vi "main.vi"() -> ()   [LabVIEW 2016]
uses:
  controls/Level2.ctl
panel:
  in  "StringArray":string[](array[string])
  in  "BooleanArray":bool[](array[boolean])
  in  "NumericArray":dbl[](array[numeric])
  in  "BigCluster":T2
  in  "Cluster":T3
  in  "String":string
  in  "Boolean":bool
  in  "Numeric":dbl
  in  "Tab Control":T4(tab)
  in  "BigCluster":T2
  in  "Cluster":T3
  in  "String":string
  in  "Boolean":bool
  in  "Numeric":dbl
  in  "Time lapse(sec)":u32
  in  "Panel Name":string
  in  "Refresh":bool
  in  "Listbox":i32(listbox)
  in  "Panel Name 2":string
  in  "Listbox 2":i32(listbox)
  in  "Run":bool
  in  "DisableListbox":i32(listbox)
  in  "MultiselectListbox":i32[](listbox)
  in  "Single Listbox":i32(listbox)
  out "Listbox Value":i32
  out "Selected Value":i32[](array[numeric])
  in  "Disabled MC Listbox":i32(listbox)
  in  "Multiselect MC Listbox":i32[](listbox)
  in  "MC Listbox":i32(listbox)
  out "MCListbox Value":i32
  out "MCL Selected Value":i32[](array[numeric])
  in  "Marksheet":string[][](table)=[["", "Class A", "Class B", "Total"], ["Biology", "10", "7", "17"], ["Chemistry", "8", "11", "19"], ["Physics", "12", "14", "26"], ["Total", "30", "32", "62"]]
  in  "Multiselect Tree":string[](tree)
  in  "Tree Control":string(tree)="Kavin"
  out "Item Tag":string
  out "Selected Tags":string[](array[string])
  out "Item Name":string
  in  "OK":bool
  in  "Stop":bool
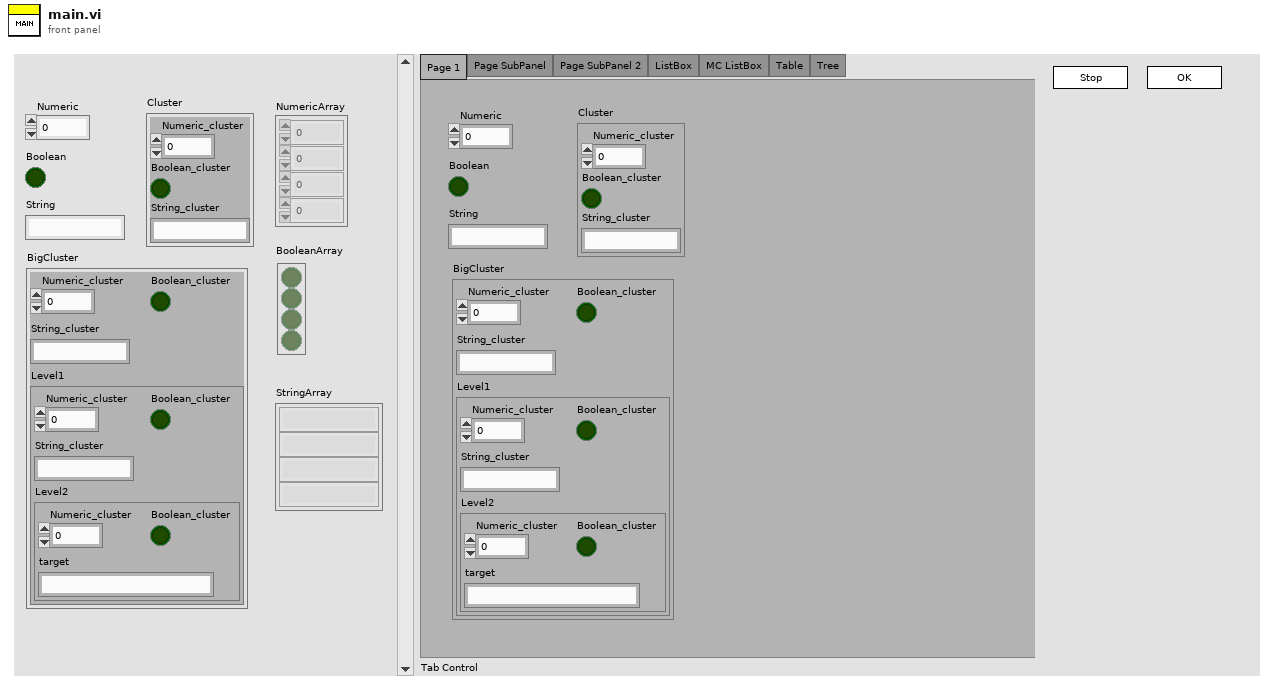
[diagram p1: front panel]
types:
  T1 = typedef "Level2.ctl" = cluster{"Numeric_cluster":dbl, "Boolean_cluster":bool, "target":string}
  T2 = cluster{"Numeric_cluster":dbl, "Boolean_cluster":bool, "String_cluster":string, "Level1":cluster{"Numeric_cluster":dbl, "Boolean_cluster":bool, "String_cluster":string, "Level2":T1}}
  T3 = cluster{"Numeric_cluster":dbl, "Boolean_cluster":bool, "String_cluster":string}
  T4 = enum32{"Page 1", "Page SubPanel", "Page SubPanel 2", "ListBox", "MC ListBox", "Table", "Tree"}
  T5 = enum32{"Invalid", "Standard", "Closed", "Hidden", "Minimized", "Maximized"}
  T6 = enum32{"invalid app kind", "Development System", "Run Time System", "Student Edition", "Embedded LabVIEW", "Evaluation", "Custom"}
  T7 = enum8{"Enabled", "Disabled", "Disabled and Grayed Out"}
  T8 = cluster{"Core":cluster{"Current VI Reference":refnum<vi>, "Close Panel on Exit?":bool}, "VI Name":string, "VI Ref":refnum<vi>, "Panel Folder Path":path, "Time lapse(sec)":u32, "Panel 2 Folder Path":path, "Panel 2 VI ref":refnum<vi>, "VI Running?":bool}
  T9 = cluster{"Current VI Reference":refnum<vi>, "Close Panel on Exit?":bool}
  T10 = enum32{"Bad", "Idle", "Run top level", "Running"}[]
  T11 = enum32{"Bad", "Idle", "Run top level", "Running"}
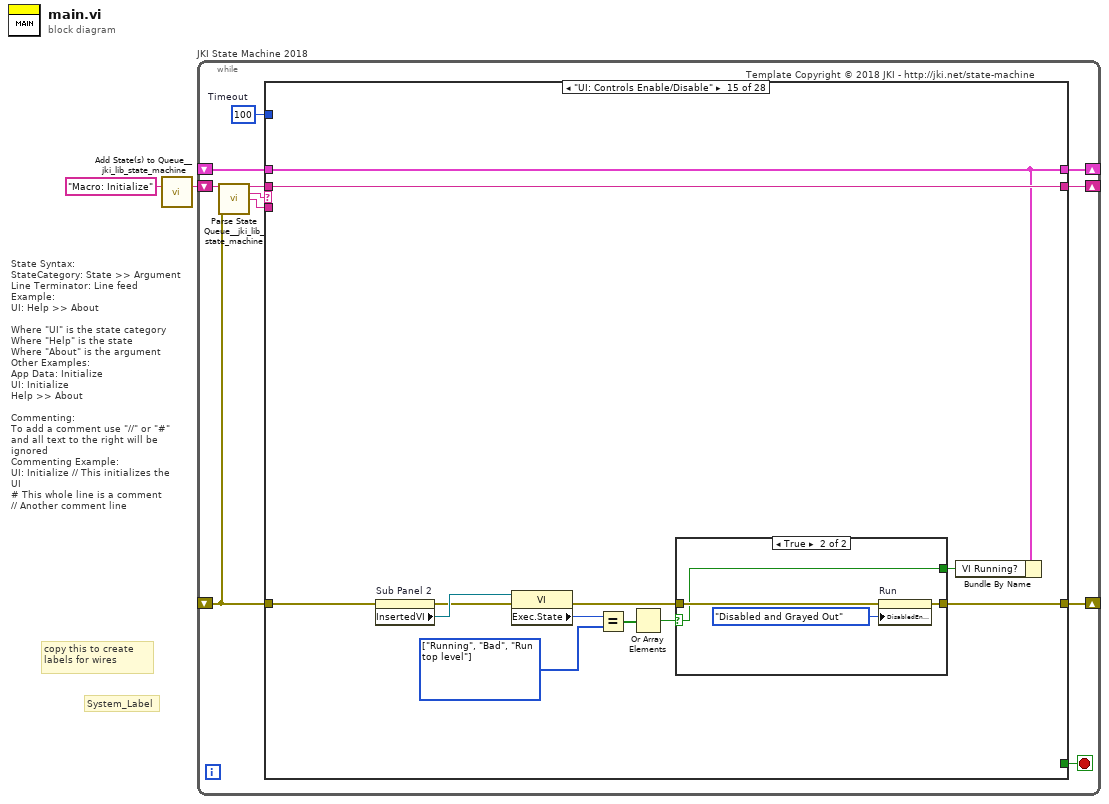
[diagram p0: block diagram]
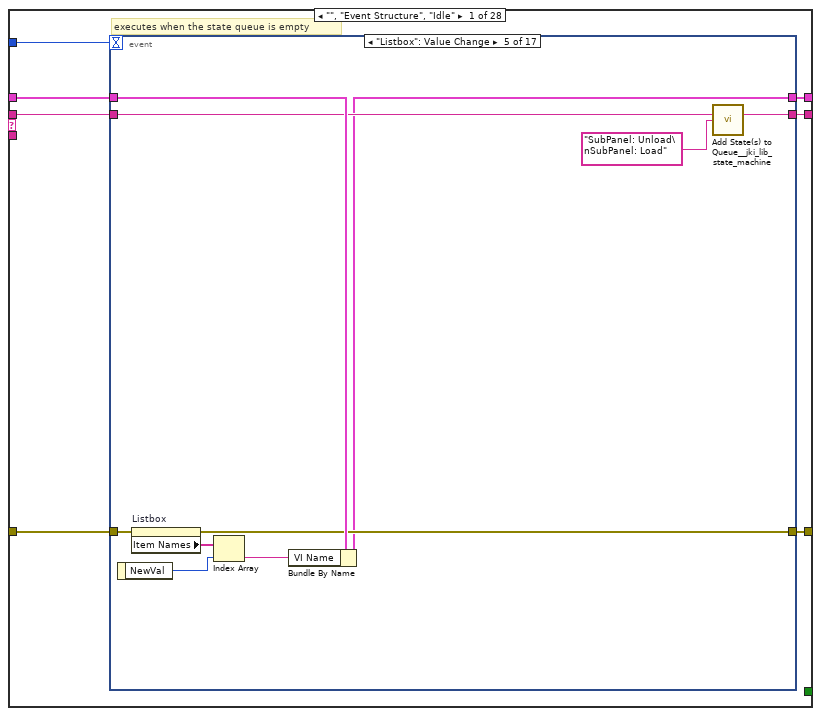
[diagram p2: hidden frame]
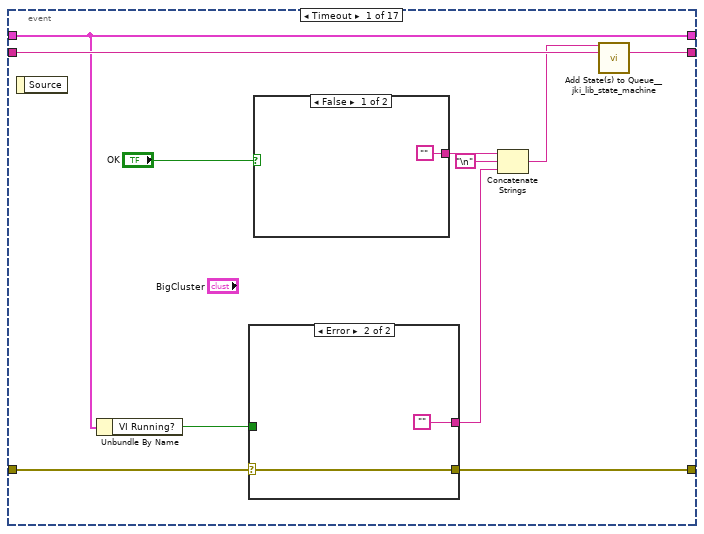
[diagram p3: hidden frame]
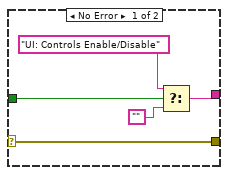
[diagram p4: hidden frame]
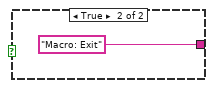
[diagram p5: hidden frame]
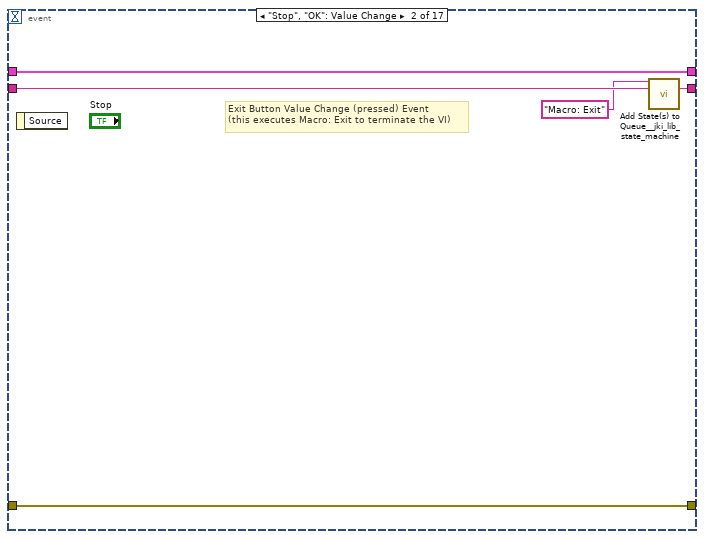
[diagram p6: hidden frame]
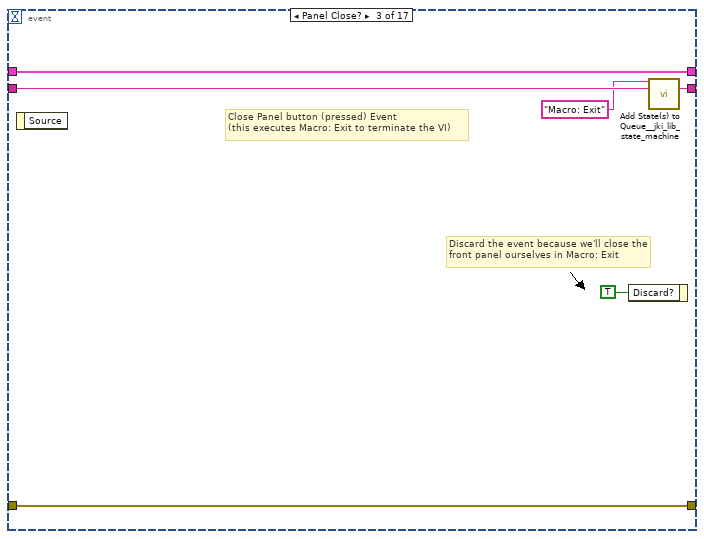
[diagram p7: hidden frame]
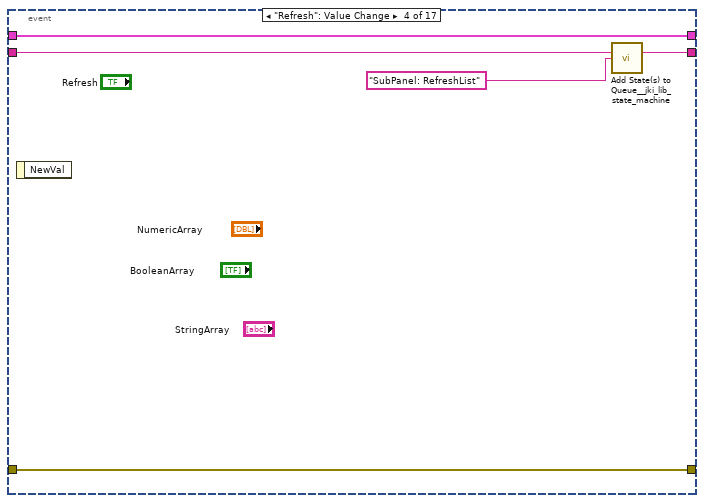
[diagram p8: hidden frame]
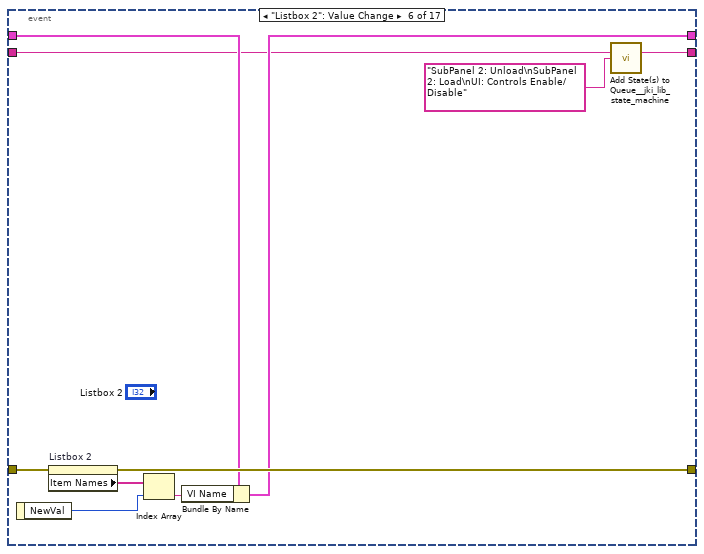
[diagram p9: hidden frame]
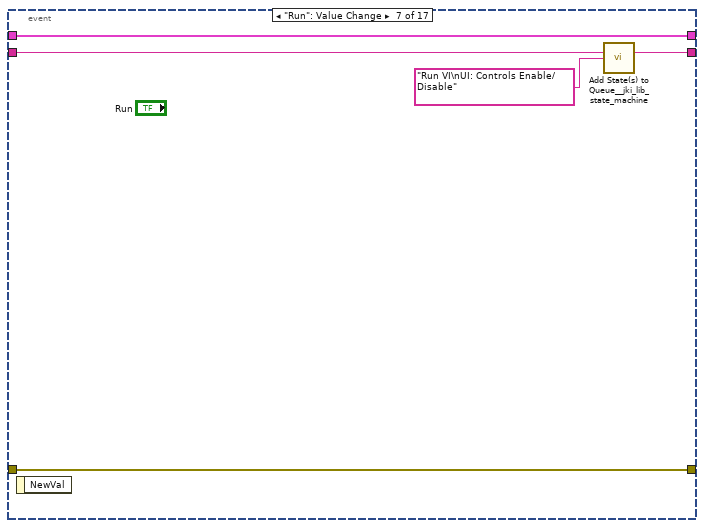
[diagram p10: hidden frame]
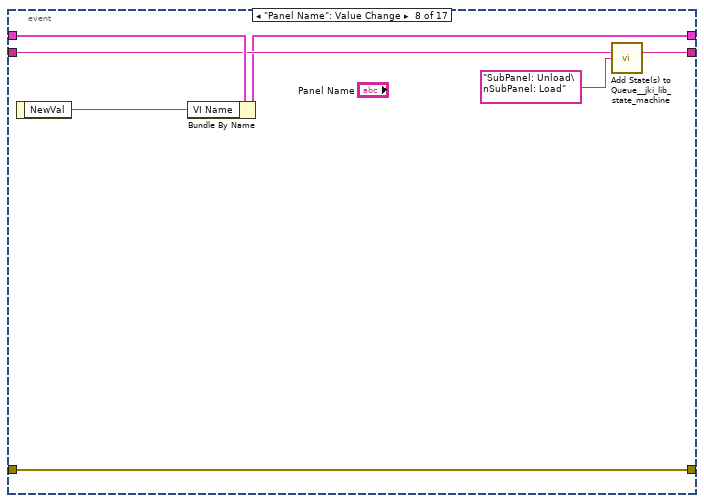
[diagram p11: hidden frame]
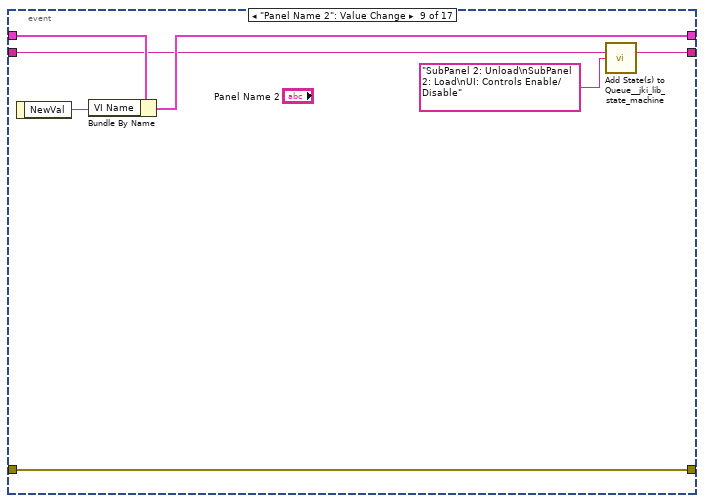
[diagram p12: hidden frame]
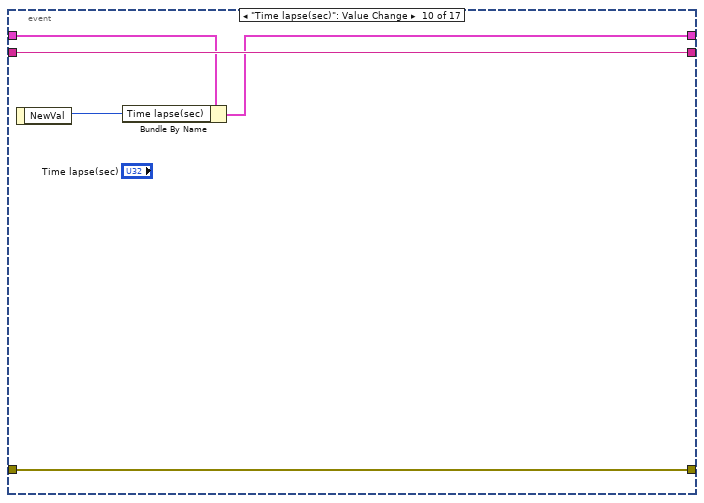
[diagram p13: hidden frame]
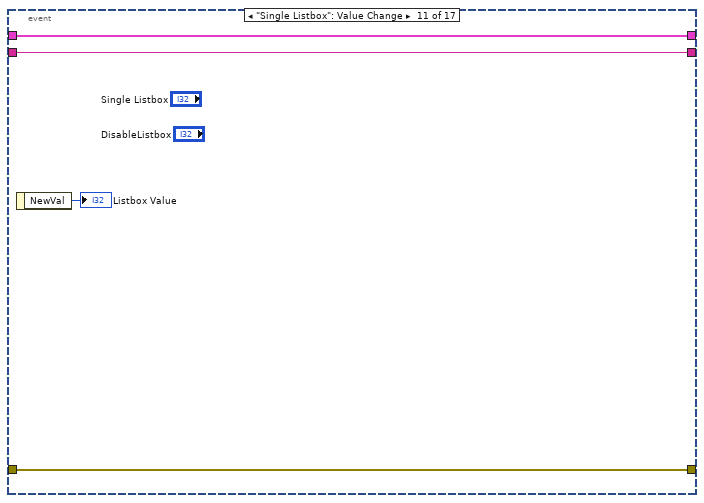
[diagram p14: hidden frame]
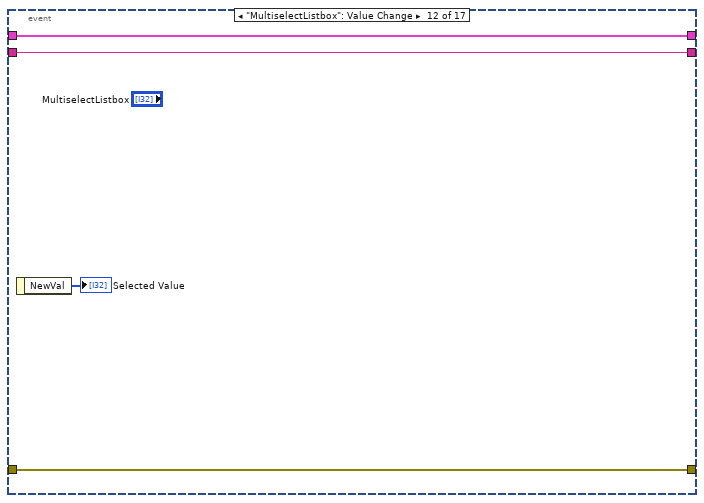
[diagram p15: hidden frame]
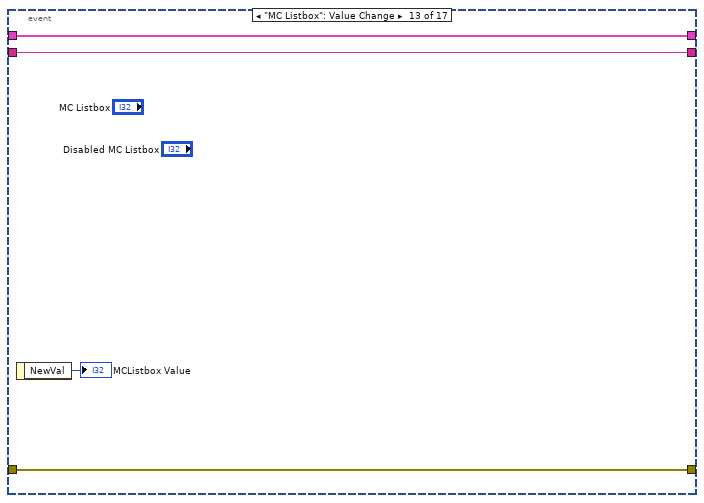
[diagram p16: hidden frame]
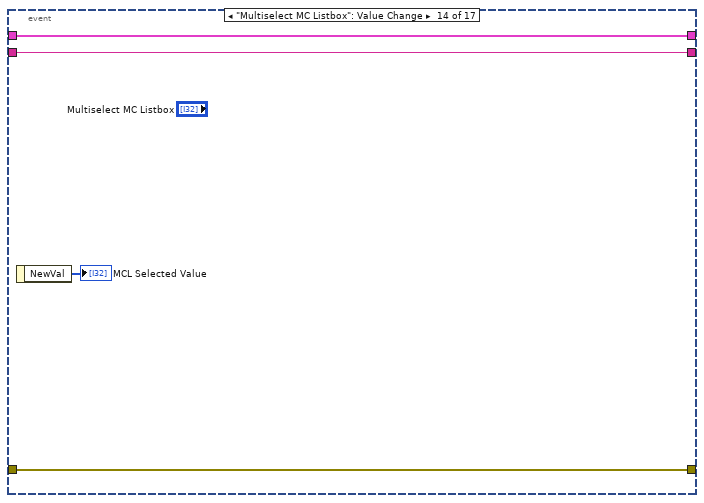
[diagram p17: hidden frame]
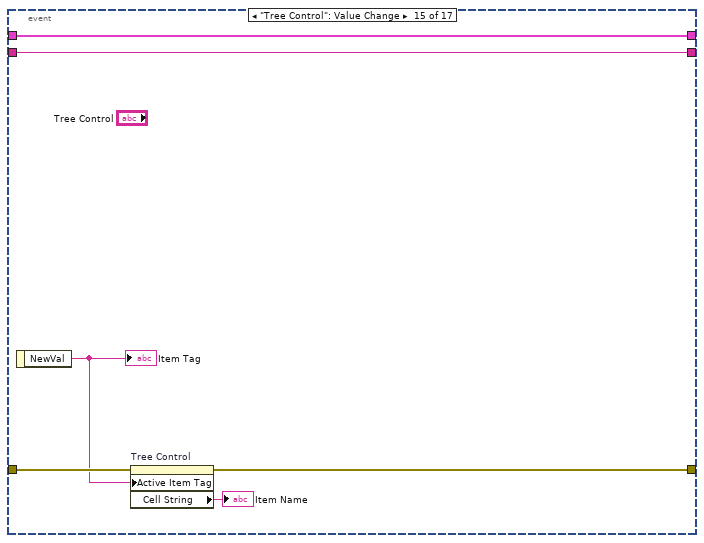
[diagram p18: hidden frame]
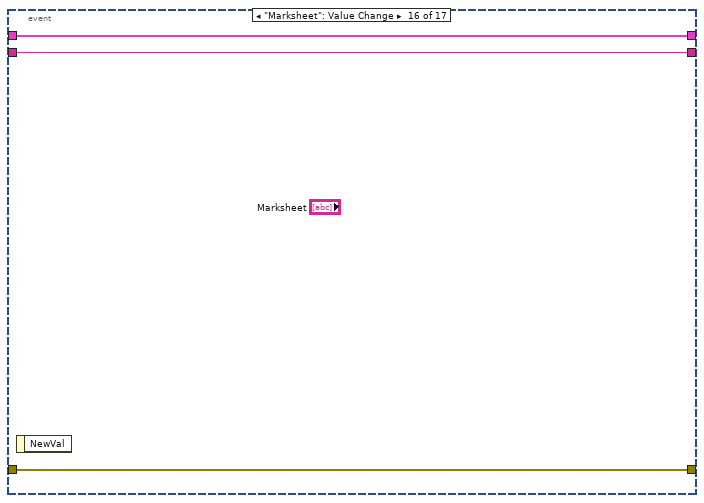
[diagram p19: hidden frame]
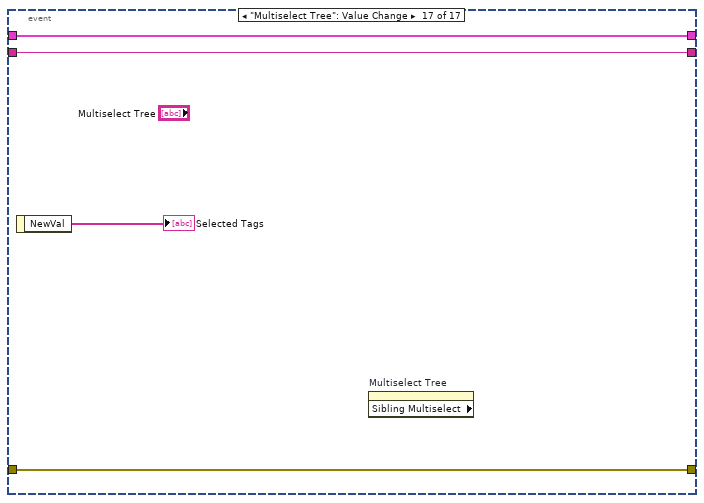
[diagram p20: hidden frame]
diagram:
  # "State Syntax:\nStateCategory: State >> Argument\nLine Terminator: Line feed\nExample:\nUI: Help >> About\n\nWhere \"UI\" is the state category\nWhere \"Help\" is the state\nWhere \"About\" is the argument\nOther Examples:\nApp Data: Initialize\nUI: Initialize\nHelp >> About\n\nCommenting:\nTo add a comment use \"//\" or \"#\" and all text to the right will be ignored\nCommenting Example:\nUI: Initialize // This initializes the UI\n# This whole line is a comment\n// Another comment line"
  # "copy this to create labels for wires"
  # "System_Label"
  n1 = call <vilib>:"Add State(s) to Queue__jki_lib_state_machine.vi"("State(s) in (\"\")"="Macro: Initialize") -> ("States Out"=w2:string)  [unwired: 14 in]
  n2 = while "JKI State Machine 2018" {
    shift-right: [w6] -> _
    shift-left: _ -> [w5]
    shift-right: [w9] -> _
    shift-left: _ -> [w3]
    shift-right: [w8] -> _
    shift-left: w2 -> [w10]
    stop <- w7 stop-if-true
    w4 = 100  # Timeout
    # "Template Copyright © 2018 JKI - http://jki.net/state-machine"
    n3 = call <vilib>:"Parse State Queue__jki_lib_state_machine.vi"("State Queue"=w10, "Error In (no error)"=w3) -> ("Remaining States"=w12:string, "Current State"=w13:string, "Arguments"=w11:string)  [unwired: 11 in]
    n4 = case shown="\"UI: Controls Enable/Disable\"" w13 {
      selector: w13 -> [_ _ w134 _ _ _ _ _ _ _ _ _ _ _ _ _ _ _ _ _ _ _ _ _ _ _ _ _]
      tunnel: w12 -> [w20 w133 w138 w159 w165 w170 w174 w194 w200 w204 w211 w217 w228 w297 w309 w321 w326 w336 w340 w354 w364 w387 w420 w434 w436 w442 w453 w457]
      tunnel: w11 -> [_ _ _ _ _ _ _ _ _ _ _ w212 w222 _ _ _ _ _ _ _ _ _ _ _ _ _ _ _]
      tunnel: w5 -> [w18 w130 w136 w155 w162 w168 w171 _ w195 w201 w209 w215 w224 w295 w298 w318 w323 w333 w337 w349 w361 w382 w418 w426 w435 w440 w450 w454]
      tunnel: [w17 w131 w140 w147 errorcluster {"status"=FALSE, "code"=0, "source"=""} ("error out") w167 w172 w175 w196 w202 w206 w213 w225 w294 w300 w319 w324 w334 w338 w342 w355 w385 w416 w428 w437 w439 w451 w455] -> w9
      tunnel: w3 -> [w16 w131 w139 w149 w161 w167 w172 w176 w197 w202 w208 w214 w226 w294 w301 w319 w324 w334 w338 w352 w357 w379 w419 w429 w437 w441 w451 w455]
      tunnel: [w19 w132 w137 w158 w164 w169 w173 w193 w199 w203 w210 w216 w227 w296 w309 w320 w325 w335 w339 w353 w363 w386 w420 w434 w436 w442 w452 w456] -> w8
      tunnel: [_ _ _ _ _ TRUE _ _ _ _ _ _ _ _ _ _ _ _ _ _ _ _ _ _ _ _ _ _] -> w7
      tunnel: [w15 w130 w136 w157 w162 w168 w171 w188 w195 w201 w209 w215 w224 w295 w298 w318 w323 w333 w337 w349 w361 w381 w418 w425 w435 w438 w450 w454] -> w6
      tunnel: w4 -> [w14 _ _ _ _ _ _ _ _ _ _ _ _ _ _ _ _ _ _ _ _ _ _ _ _ _ _ _]
      frame "", "Event Structure", "Idle" {
        # "executes when the state queue is empty"
        n5 = event shown="[4] \"Listbox\": Value Change" {
          selector: _ -> [_ _ _ _ _ _ _ _ _ _ _ _ _ _ _ _ _]
          dyn-events: _ -> [_ _ _ _ _ _ _ _ _ _ _ _ _ _ _ _ _]
          timeout: w14 -> [_ _ _ _ _ _ _ _ _ _ _ _ _ _ _ _ _]
          tunnel: w20 -> [w31 w45 w51 w54 w65 w68 w79 w87 w90 w100 w104 w108 w112 w116 w122 w125 w129]
          tunnel: [w30 w44 w50 w53 w64 w67 w78 w86 w89 w100 w104 w108 w112 w116 w122 w125 w129] -> w19
          tunnel: w18 -> [w28 w42 w48 w55 w66 w71 w80 w88 w93 w97 w102 w106 w110 w114 w121 w123 w127]
          tunnel: [w21 w43 w49 w56 w61 w74 w81 w84 w95 w99 w103 w107 w111 w115 w119 w124 w128] -> w17
          tunnel: w16 -> [w22 w43 w49 w56 w62 w75 w81 w84 w95 w99 w103 w107 w111 w115 w120 w124 w128]
          tunnel: [w28 w42 w48 w55 w58 w70 w80 w82 w92 w96 w102 w106 w110 w114 w121 w123 w127] -> w15
          event Timeout {
            n6 = event-data() -> ()  [unwired: 1 in, 1 out]
            n7 = Unbundle By Name(w28) -> ("VI Running?"=w27:bool)
            n8 = case shown="Error" w22 {
              selector: w22 -> [w32 w37]
              tunnel: [w33 ""] -> w26
              tunnel: w27 -> [w36 _]
              tunnel: [w32 w37] -> w21
              frame No Error {
                n9 = Select(t="UI: Controls Enable/Disable", s=w36, f="") -> (s? t:f=w33:string)
              }
              frame Error {
              }
            }
            n10 = case shown="False" "OK" {
              tunnel: ["" "Macro: Exit"] -> w25
              frame False {
              }
              frame True {
              }
            }
            n11 = Concatenate Strings(w25, "\n", w26) -> (w23:string)
            n12 = call <vilib>:"Add State(s) to Queue__jki_lib_state_machine.vi"("State(s) in Front (\"\")"=w23, "State(s) in (\"\")"=w31) -> ("States Out"=w30:string)  [unwired: 13 in]
          }
          event "Stop", "OK": Value Change {
            # "Exit Button Value Change (pressed) Event\n(this executes Macro: Exit to terminate the VI)"
            n13 = event-data() -> ()  [unwired: 1 in, 1 out]
            n14 = call <vilib>:"Add State(s) to Queue__jki_lib_state_machine.vi"("State(s) in Front (\"\")"="Macro: Exit", "State(s) in (\"\")"=w45) -> ("States Out"=w44:string)  [unwired: 13 in]
          }
          event Panel Close? {
            # "Discard the event because we'll close the front panel ourselves in Macro: Exit"
            # "Close Panel button (pressed) Event\n(this executes Macro: Exit to terminate the VI)"
            n15 = event-data() -> ()  [unwired: 1 in, 1 out]
            n16 = event-data("Discard?"=TRUE) -> ()  [unwired: 1 in, 1 out]
            n17 = call <vilib>:"Add State(s) to Queue__jki_lib_state_machine.vi"("State(s) in Front (\"\")"="Macro: Exit", "State(s) in (\"\")"=w51) -> ("States Out"=w50:string)  [unwired: 13 in]
          }
          event "Refresh": Value Change {
            n18 = event-data() -> ()  [unwired: 1 in, 1 out]
            n19 = call <vilib>:"Add State(s) to Queue__jki_lib_state_machine.vi"("State(s) in (\"\")"=w54, "State(s) at Back (\"\")"="SubPanel: RefreshList") -> ("States Out"=w53:string)  [unwired: 13 in]
          }
          event "Listbox": Value Change {
            n20 = event-data() -> ("NewVal"=w59:i32)  [unwired: 1 in]
            n21 = property on="Listbox" class="LstBox (strict)"(error in=w62) -> (error out=w61:errorcluster, "Item Names"=w60:string[])  [unwired: 1 in, 1 out]
            n22 = Index Array(array=w60, index=w59) -> (element=w57:string)
            n23 = Bundle By Name(cluster=w66, "VI Name"=w57) -> (w58:T8)
            n24 = call <vilib>:"Add State(s) to Queue__jki_lib_state_machine.vi"("State(s) in (\"\")"=w65, "State(s) at Back (\"\")"="SubPanel: Unload\nSubPanel: Load") -> ("States Out"=w64:string)  [unwired: 13 in]
          }
          event "Listbox 2": Value Change {
            n25 = event-data() -> ("NewVal"=w73:i32)  [unwired: 1 in]
            n26 = property on="Listbox 2" class="LstBox (strict)"(error in=w75) -> (error out=w74:errorcluster, "Item Names"=w76:string[])  [unwired: 1 in, 1 out]
            n27 = Index Array(array=w76, index=w73) -> (element=w72:string)
            n28 = Bundle By Name(cluster=w71, "VI Name"=w72) -> (w70:T8)
            n29 = call <vilib>:"Add State(s) to Queue__jki_lib_state_machine.vi"("State(s) in (\"\")"=w68, "State(s) at Back (\"\")"="SubPanel 2: Unload\nSubPanel 2: Load\nUI: Controls Enable/Disable") -> ("States Out"=w67:string)  [unwired: 13 in]
          }
          event "Run": Value Change {
            n30 = event-data() -> ()  [unwired: 1 in, 1 out]
            n31 = call <vilib>:"Add State(s) to Queue__jki_lib_state_machine.vi"("State(s) in (\"\")"=w79, "State(s) at Back (\"\")"="Run VI\nUI: Controls Enable/Disable" ("State(s) at Back (\"\")")) -> ("States Out"=w78:string)  [unwired: 13 in]
          }
          event "Panel Name": Value Change {
            n32 = event-data() -> ("NewVal"=w83:string)  [unwired: 1 in]
            n33 = Bundle By Name(cluster=w88, "VI Name"=w83) -> (w82:T8)
            n34 = call <vilib>:"Add State(s) to Queue__jki_lib_state_machine.vi"("State(s) in (\"\")"=w87, "State(s) at Back (\"\")"="SubPanel: Unload\nSubPanel: Load") -> ("States Out"=w86:string)  [unwired: 13 in]
          }
          event "Panel Name 2": Value Change {
            n35 = event-data() -> ("NewVal"=w94:string)  [unwired: 1 in]
            n36 = Bundle By Name(cluster=w93, "VI Name"=w94) -> (w92:T8)
            n37 = call <vilib>:"Add State(s) to Queue__jki_lib_state_machine.vi"("State(s) in (\"\")"=w90, "State(s) at Back (\"\")"="SubPanel 2: Unload\nSubPanel 2: Load\nUI: Controls Enable/Disable") -> ("States Out"=w89:string)  [unwired: 13 in]
          }
          event "Time lapse(sec)": Value Change {
            n38 = event-data() -> ("NewVal"=w98:u32)  [unwired: 1 in]
            n39 = Bundle By Name(cluster=w97, "Time lapse(sec)"=w98) -> (w96:T8)
          }
          event "Single Listbox": Value Change {
            n40 = event-data() -> ("NewVal"=→"Listbox Value":i32)  [unwired: 1 in]
          }
          event "MultiselectListbox": Value Change {
            n41 = event-data() -> ("NewVal"=→"Selected Value":i32[])  [unwired: 1 in]
          }
          event "MC Listbox": Value Change {
            n42 = event-data() -> ("NewVal"=→"MCListbox Value":i32)  [unwired: 1 in]
          }
          event "Multiselect MC Listbox": Value Change {
            n43 = event-data() -> ("NewVal"=→"MCL Selected Value":i32[])  [unwired: 1 in]
          }
          event "Tree Control": Value Change {
            n44 = event-data() -> ("NewVal"=w118:string)  [unwired: 1 in]
            "Item Tag" <- w118
            n45 = property on="Tree Control" class="Tree (strict)"(error in=w120, "Active Item Tag"=w118) -> (error out=w119:errorcluster, "Cell String"=→"Item Name":string)  [unwired: 1 in, 1 out]
          }
          event "Marksheet": Value Change {
            n46 = event-data() -> ()  [unwired: 1 in, 1 out]
          }
          event "Multiselect Tree": Value Change {
            n47 = event-data() -> ("NewVal"=→"Selected Tags":string[])  [unwired: 1 in]
            n48 = property on="Multiselect Tree" class="Tree (strict)" props=["Sibling Multiselect"]() -> ()  [unwired: 2 in, 3 out]
          }
        }
      }
      frame "---------- Core ----------" {
        # "Do not put any code in this frame.\n(it is a separator no-op)"
        n49 = call <vilib>:"Add State(s) to Queue__jki_lib_state_machine.vi"("State(s) in (\"\")"=w133) -> ("States Out"=w132:string)  [unwired: 14 in]
      }
      frame Default {
        w143 = 42 items=["No error", "Argument error", "Memory is full", "Out of zone", "End of file", "File already open", "Generic file I/O error", "File not found", "File permission error", "Disk is full", "Duplicate path", "Too many files open", "System feature not enabled", "Resource file not found", "Cannot add resource", "Resource not found", "Image not found", "Image memory error", "Pen does not exist", "Config type invalid", "Config token not found", "Config parse error", "Config memory error", "Bad external code format", "Bad external code offset", "External code not present", "Null window", "Destroy window error", "Null menu", "Print aborted", "Bad print record", "Print driver error", "Windows error during printing", "Memory error during printing", "Print dialog error", "Generic print error", "Invalid device refnum", "Device not found", "Device parameter error", "Device unit error", "Cannot open device", "Device call aborted", "Generic error", "Cancelled by user", "Object ID too low", "Object ID too high", "Object not in heap", "Unknown heap", "Unknown object (invalid DefProc)", "Unknown object (DefProc not in table)", "Message out of range", "Invalid (null) method", "Unknown message", "Manager call not supported", "Bad address", "Network operation in progress", "Network operation timed out", "Connection is busy", "Network attribute not supported", "Network error", "Address in use", "System out of memory", "Connection aborted", "Connection refused", "Not connected", "Already connected", "Connection closed", "Initialization error (interapplication manager)", "Bad occurrence", "Wait on unbound occurrence handler", "Occurrence queue overflow", "Datalog type conflict", "Unused", "Unrecognized type (interapplication manager)", "Memory corrupt", "Failed to make temporary DLL", "Old CIN version", "Drag socket not found", "Failed to load drop-object", "Failed to register OLE object", "Failed to release OLE object", "Format specifier type mismatch", "Unknown format specifier", "Too few format specifiers", "Too many format specifiers", "Scan failed", "Newer CIN version", "Error converting to variant", "Runtime menu error", "Password tampered", "Variant attribute not found", "Incompatible variant data type", "Event data is not available", "Event Store is not present", "Occurrence is not found", "Event Queue is not created", "Event info is not available", "Refnum passed is NULL", "Error retrieving Class GUID", "Error retrieving CoClass GUID", "Error retrieving TypeLib GUID.", "Bad built application magic bytes.", "Specific driver is different from the specific driver associated with the Logical Name.", "There is no session opened to the class driver.", "Max Error", "MAX - Error with config objects", "MAX - Error loading configuration", "MAX - Group not supported"]
        # "Current State"
        # "Do not delete, rename, or modify this frame.\n(this is used to capture unhandled states and typos)"
        # "Handle mistyped state name (developer tool)"
        n50 = Format Into String(format string="Software Exception: Unhandled State \"%s\"." ("message"), error in=w139, w134) -> (resulting string=w142:string, error out=w141:errorcluster)  [unwired: 1 in]
        n51 = call <vilib>:"Error Cluster From Error Code.vi"("show call chain? (False)"=TRUE, "error in (no error)"=w141, "error message (\"\")"=w142, "error code (0)"=w143) -> ("error out"=w140:errorcluster)  [unwired: 5 in]
        n52 = call <vilib>:"Add State(s) to Queue__jki_lib_state_machine.vi"("State(s) in (\"\")"=w138) -> ("States Out"=w137:string)  [unwired: 14 in]
      }
      frame "Initialize Core Data" {
        # "Do not delete, rename, or modify this frame.\n(this is used to determine panel behavior on exit)"
        # "originally closed?"
        # "exe?"
        # "If panel starts closed or is an EXE, then close it when we exit"
        n53 = property class="VI"(error in=w149) -> (error out=w148:errorcluster, "FP.State"=w152:T5)  [unwired: 1 in, 1 out]
        n54 = property class="App"(error in=w148) -> (error out=w147:errorcluster, "App.Kind"=w146:T6)  [unwired: 1 in, 1 out]
        n55 = control-ref of="Current VI Reference"() -> (w153:refnum<vi>)
        n56 = Equal?(x=w152, y=T5."Closed" ("Front Panel Window:State")) -> (x = y?=w150:bool)
        n57 = Equal?(x=T6."Run Time System" ("Application:Kind"), y=w146) -> (x = y?=w156:bool)
        n58 = Or(x=w150, y=w156) -> (x .or. y?=w154:bool)
        n59 = Bundle By Name(cluster=w155, "Core.Current VI Reference"=w153, "Core.Close Panel on Exit?"=w154) -> (w157:T8)
        n60 = call <vilib>:"Add State(s) to Queue__jki_lib_state_machine.vi"("State(s) in (\"\")"=w159) -> ("States Out"=w158:string)  [unwired: 14 in]
      }
      frame "Error Handler" {
        # "Unhandled Error -- Display it"
        # "Handle any errors here.\nYou can also output any states to clean-up after errors occur"
        # "Clear error"
        n61 = call <vilib>:"General Error Handler.vi"("error in (no error)"=w161) -> ()  [unwired: 10 in, 5 out]
        n62 = call <vilib>:"Add State(s) to Queue__jki_lib_state_machine.vi"("State(s) in Front (\"\")"="/* Post Error States", "State(s) in (\"\")"=w165) -> ("States Out"=w164:string)  [unwired: 13 in]
      }
      frame "Exit" {
        # "Do not put any code in this frame.\n(No errors that occur here will be handled.)"
        n63 = call <vilib>:"Add State(s) to Queue__jki_lib_state_machine.vi"("State(s) in (\"\")"=w170) -> ("States Out"=w169:string)  [unwired: 14 in]
      }
      frame "---------- Data ----------" {
        # "Do not put any code in this frame.\n(It is a separator no-op. You can make a copy of this frame to create a new Data frame)"
        n64 = call <vilib>:"Add State(s) to Queue__jki_lib_state_machine.vi"("State(s) in (\"\")"=w174) -> ("States Out"=w173:string)  [unwired: 14 in]
      }
      frame "Data: Initialize" {
        w182 = FALSE  # VI Running?
        w183 = refnum<vi> refnum  # Panel 2 VI ref
        w185 = path ""  # Panel 2 Folder Path
        w186 = u32 0  # Time lapse(sec)
        w187 = refnum<vi> refnum  # VI Ref
        w189 = path ""  # Panel Folder Path
        w190 = T9 {"Current VI Reference"=refnum, "Close Panel on Exit?"=FALSE}  # Core
        w191 = ""  # VI Name
        # "Initialize the shift-register data, here.\n(data names are defined by what you wire into the bundle function)"
        n65 = vi-ref "_Template.vi"() -> (w179:refnum<vi>)
        n66 = property class="VI"(reference=w179, error in=w176) -> (error out=w175:errorcluster, "Path"=w178:path)  [unwired: 1 out]
        n67 = Strip Path(path=w178) -> (stripped path=w177:path)  [unwired: 1 out]
        n68 = Bundle("Core"=w190, "VI Name"=w191, "VI Ref"=w187, "Panel Folder Path"=w189, "Time lapse(sec)"=w186, "Panel 2 Folder Path"=w185, "Panel 2 VI ref"=w183, "VI Running?"=w182) -> (w192:T8)  [unwired: 1 in]
        n69 = Strip Path(path=w177) -> (stripped path=w181:path)  [unwired: 1 out]
        n70 = Build Path(base path=w181, name or relative path="ExecPanels") -> (appended path=w184:path)
        n71 = Bundle By Name(cluster=w192, "Panel Folder Path"=w177, "Panel 2 Folder Path"=w184) -> (w188:T8)
        n72 = call <vilib>:"Add State(s) to Queue__jki_lib_state_machine.vi"("State(s) in (\"\")"=w194) -> ("States Out"=w193:string)  [unwired: 14 in]
      }
      frame "Data: Cleanup" {
        # "Cleanup any data and references, here.\n(this is called automatically, by the Macro: Exit)"
        n73 = Unbundle By Name(w195) -> ("Core.Current VI Reference"=w198:refnum<vi>)
        n74 = Close Reference(reference=w198, error in (no error)=w197) -> (error out=w196:errorcluster)
        n75 = call <vilib>:"Add State(s) to Queue__jki_lib_state_machine.vi"("State(s) in (\"\")"=w200) -> ("States Out"=w199:string)  [unwired: 14 in]
      }
      frame "---------- UI ----------" {
        # "Do not put any code in this frame.\n(It is a separator no-op. You can make a copy of this frame to create a new UI frame)"
        n76 = call <vilib>:"Add State(s) to Queue__jki_lib_state_machine.vi"("State(s) in (\"\")"=w204) -> ("States Out"=w203:string)  [unwired: 14 in]
      }
      frame "UI: Initialize" {
        # "Initialize the User Interface, here.\n(this is called automatically, by the Macro: Init)"
        n77 = invoke class="VI" method="Default Vals.Reinit All"(error in=w208) -> (error out=w207:errorcluster)  [unwired: 2 in, 2 out]
        n78 = property on="Run" class="Bool"(error in=w207, "DisabledEnum"=T7."Disabled and Grayed Out" ("Disabled")) -> (error out=w206:errorcluster)  [unwired: 1 in, 1 out]
        n79 = call <vilib>:"Add State(s) to Queue__jki_lib_state_machine.vi"("State(s) in (\"\")"=w211) -> ("States Out"=w210:string)  [unwired: 14 in]
      }
      frame "UI: Cursor Set" {
        # "Argument"
        # "Set and Unset Cursor Busy.\n(Usage: \"UI: Cursor Set >> Busy|Idle\")"
        n80 = case shown="\"Idle\", Default" w212 {
          tunnel: w214 -> [w219 w221]
          tunnel: [w218 w220] -> w213
          frame "Idle", Default {
            n81 = call <vilib>:"Unset Busy.vi"("error in (no error)"=w219) -> ("error out"=w218:errorcluster)  [unwired: 10 in]
          }
          frame "Busy" {
            n82 = call <vilib>:"Set Busy.vi"("error in (no error)"=w221) -> ("error out"=w220:errorcluster)  [unwired: 9 in, 1 out]
          }
        }
        n83 = call <vilib>:"Add State(s) to Queue__jki_lib_state_machine.vi"("State(s) in (\"\")"=w217) -> ("States Out"=w216:string)  [unwired: 14 in]
      }
      frame "UI: Front Panel State" {
        # "Argument"
        # "Set Front Panel Open or Closed\n(Usage: \"UI: Front Panel State >> Open|Close\")"
        n84 = Unbundle By Name(w224) -> ("Core.Current VI Reference"=w223:refnum<vi>)
        n85 = case shown="\"Close\", \"Closed\"" w222 {
          tunnel: w226 -> [w234 w249 w260 w273 w286]
          tunnel: [w236 w250 w262 w275 w288] -> w225
          tunnel: w223 -> [w235 w247 w261 w274 w287]
          frame "Open", "Standard", Default {
            w229 = T5."Standard" ("State")
            n86 = property class="VI"(reference=w235, error in=w234) -> (reference out=w232:refnum<vi>, error out=w233:errorcluster, "FP.State"=w231:T5)
            n87 = Not Equal?(x=w231, y=w229) -> (x != y?=w230:bool)
            n88 = case shown="True" w230 {
              tunnel: [w240 w242] -> w236
              tunnel: w233 -> [w239 w242]
              tunnel: w232 -> [w238 _]
              tunnel: w229 -> [w237 _]
              frame True {
                n89 = invoke class="VI" method="FP.Open"(reference=w238, error in=w239, "Activate"=TRUE, "State"=w237) -> (error out=w240:errorcluster)  [unwired: 1 in, 4 out]
              }
              frame False {
              }
            }
          }
          frame "Close", "Closed" {
            n90 = property class="VI"(reference=w247, error in=w249) -> (reference out=w246:refnum<vi>, error out=w248:errorcluster, "FP.State"=w244:T5)
            n91 = Not Equal?(x=w244, y=T5."Closed" ("Front Panel Window:State")) -> (x != y?=w243:bool)
            n92 = case shown="True" w243 {
              tunnel: [w251 w254] -> w250
              tunnel: w248 -> [w251 w253]
              tunnel: w246 -> [_ w252]
              frame False {
              }
              frame True {
                n93 = invoke class="VI" method="FP.Close"(reference=w252, error in=w253) -> (error out=w254:errorcluster)  [unwired: 1 in, 2 out]
              }
            }
          }
          frame "Hidden", "Hide" {
            w255 = T5."Hidden" ("State")
            n94 = property class="VI"(reference=w261, error in=w260) -> (reference out=w258:refnum<vi>, error out=w259:errorcluster, "FP.State"=w257:T5)
            n95 = Not Equal?(x=w257, y=w255) -> (x != y?=w256:bool)
            n96 = case shown="True" w256 {
              tunnel: [w266 w267] -> w262
              tunnel: w259 -> [w265 w267]
              tunnel: w258 -> [w264 _]
              tunnel: w255 -> [w263 _]
              frame True {
                n97 = invoke class="VI" method="FP.Open"(reference=w264, error in=w265, "State"=w263) -> (error out=w266:errorcluster)  [unwired: 2 in, 4 out]
              }
              frame False {
              }
            }
          }
          frame "Minimize", "Minimized" {
            w268 = T5."Minimized" ("State")
            n98 = property class="VI"(reference=w274, error in=w273) -> (reference out=w271:refnum<vi>, error out=w272:errorcluster, "FP.State"=w270:T5)
            n99 = Not Equal?(x=w270, y=w268) -> (x != y?=w269:bool)
            n100 = case shown="True" w269 {
              tunnel: [w279 w280] -> w275
              tunnel: w272 -> [w278 w280]
              tunnel: w271 -> [w277 _]
              tunnel: w268 -> [w276 _]
              frame True {
                n101 = invoke class="VI" method="FP.Open"(reference=w277, error in=w278, "State"=w276) -> (error out=w279:errorcluster)  [unwired: 2 in, 4 out]
              }
              frame False {
              }
            }
          }
          frame "Maximize", "Maximized" {
            w281 = T5."Maximized" ("State")
            n102 = property class="VI"(reference=w287, error in=w286) -> (reference out=w284:refnum<vi>, error out=w285:errorcluster, "FP.State"=w283:T5)
            n103 = Not Equal?(x=w283, y=w281) -> (x != y?=w282:bool)
            n104 = case shown="True" w282 {
              tunnel: [w292 w293] -> w288
              tunnel: w285 -> [w291 w293]
              tunnel: w284 -> [w290 _]
              tunnel: w281 -> [w289 _]
              frame True {
                n105 = invoke class="VI" method="FP.Open"(reference=w290, error in=w291, "State"=w289) -> (error out=w292:errorcluster)  [unwired: 2 in, 4 out]
              }
              frame False {
              }
            }
          }
        }
        n106 = call <vilib>:"Add State(s) to Queue__jki_lib_state_machine.vi"("State(s) in (\"\")"=w228) -> ("States Out"=w227:string)  [unwired: 14 in]
      }
      frame "UI: Update" {
        n107 = call <vilib>:"Add State(s) to Queue__jki_lib_state_machine.vi"("State(s) in (\"\")"=w297) -> ("States Out"=w296:string)  [unwired: 14 in]
      }
      frame "UI: Controls Enable/Disable" {
        w305 = T10 [enum."Running", enum."Bad", enum."Run top level"] items=["Bad", "Idle", "Run top level", "Running"] ("y")
        n108 = property on="Sub Panel 2" class="SubPnl"(error in=w301) -> (error out=w307:errorcluster, "InsertedVI"=w308:refnum<vi>)  [unwired: 1 in, 1 out]
        n109 = property class="VI"(reference=w308, error in=w307) -> (error out=w302:errorcluster, "Exec.State"=w306:T11)  [unwired: 1 out]
        n110 = Equal?(x=w306, y=w305) -> (x = y?=w304:bool[])
        n111 = Or Array Elements(Boolean array=w304) -> (logical OR=w303:bool)
        n112 = case shown="True" w303 {
          selector: w303 -> [w310 w314]
          tunnel: w302 -> [w312 w317]
          tunnel: [w311 w315] -> w300
          tunnel: [w310 w314] -> w299
          frame False {
            n113 = property on="Run" class="Bool"(error in=w312, "DisabledEnum"=T7."Enabled" ("Disabled")) -> (error out=w311:errorcluster)  [unwired: 1 in, 1 out]
          }
          frame True {
            n114 = property on="Run" class="Bool"(error in=w317, "DisabledEnum"=T7."Disabled and Grayed Out" ("Disabled")) -> (error out=w315:errorcluster)  [unwired: 1 in, 1 out]
          }
        }
        n115 = Bundle By Name(cluster=w298, "VI Running?"=w299) -> ()  [unwired: 1 out]
      }
      frame "---------- Macro ----------" {
        # "Do not put any code in this frame.\n(It is a separator no-op. You can make a copy of this frame to create a new Macro frame)"
        n116 = call <vilib>:"Add State(s) to Queue__jki_lib_state_machine.vi"("State(s) in (\"\")"=w321) -> ("States Out"=w320:string)  [unwired: 14 in]
      }
      frame "Macro: Initialize" {
        w322 = "Data: Initialize\nInitialize Core Data\nUI: Initialize\nUI: Front Panel State >> Open\n# Custom States\nSubPanel: RefreshList"  # Data: Initialize Initialize Core Data UI: Initialize UI: Front Panel State >> Open # Custom States SubPanel: RefreshList
        # "Initialization Macro\n(This is called once, when the VI starts)"
        n117 = call <vilib>:"Add State(s) to Queue__jki_lib_state_machine.vi"("State(s) in Front (\"\")"=w322, "State(s) in (\"\")"=w326) -> ("States Out"=w325:string)  [unwired: 13 in]
      }
      frame "Macro: Exit" {
        # "Exit Macro\n(This is called once, when the VI exits)"
        n118 = Unbundle By Name(w333) -> ("Core.Close Panel on Exit?"=w332:bool)
        n119 = Select(t="UI: Front Panel State >> Close", s=w332, f="") -> (s? t:f=w329:string)
        n120 = call <vilib>:"Add State(s) to Queue__jki_lib_state_machine.vi"("State(s) in (\"\")"=w329, "State(s) at Back (\"\")"="SubPanel: Unload\nSubPanel 2: Unload\nData: Cleanup\nExit") -> ("States Out"=w327:string)  [unwired: 13 in]
        n121 = call <vilib>:"Add State(s) to Queue__jki_lib_state_machine.vi"("State(s) in Front (\"\")"=w327, "State(s) in (\"\")"=w336) -> ("States Out"=w335:string)  [unwired: 13 in]
      }
      frame "---------- SubPanel ----------" {
        # "Template Separator\n(You can make a copy of, or modify, this frame)"
        n122 = call <vilib>:"Add State(s) to Queue__jki_lib_state_machine.vi"("State(s) in (\"\")"=w340) -> ("States Out"=w339:string)  [unwired: 14 in]
      }
      frame "SubPanel: RefreshList" {
        w341 = -1 ("Listbox")
        n123 = Unbundle By Name(w349) -> ("Panel 2 Folder Path"=w344:path, "Panel Folder Path"=w348:path)
        n124 = List Folder(path=w348, pattern="*.vi", error in=w352) -> (filenames=w350:string[], error out=w351:errorcluster)  [unwired: 1 in, 2 out]
        n125 = property on="Listbox" class="LstBox (strict)"(error in=w351, "Item Names"=w350, "Value"=w341) -> (error out=w343:errorcluster)  [unwired: 1 in, 1 out]
        n126 = List Folder(path=w344, error in=w343) -> (filenames=w346:string[], error out=w345:errorcluster)  [unwired: 2 in, 2 out]
        n127 = property on="Listbox 2" class="LstBox (strict)"(error in=w345, "Item Names"=w346, "Value"=w341) -> (error out=w342:errorcluster)  [unwired: 1 in, 1 out]
        n128 = call <vilib>:"Add State(s) to Queue__jki_lib_state_machine.vi"("State(s) in (\"\")"=w354) -> ("States Out"=w353:string)  [unwired: 14 in]
      }
      frame "SubPanel: Unload" {
        n129 = invoke on="Sub Panel" class="SubPnl" method="Remove VI"(error in=w357) -> (error out=w362:errorcluster)  [unwired: 2 in, 2 out]
        n130 = call <vilib>:"Clear Errors.vi"("error in (no error)"=w362) -> ("error out"=w356:errorcluster)  [unwired: 5 in, 1 out]
        n131 = Unbundle By Name(w361) -> ("VI Ref"=w360:refnum<vi>)
        n132 = Not A Number/Path/Refnum?(number/path/refnum=w360) -> (NaN/Path/Refnum?=w359:bool)
        n133 = case shown="False" w359 {
          tunnel: w356 -> [w373 w374]
          tunnel: [w369 w374] -> w358
          tunnel: w360 -> [w370 _]
          frame False {
            n134 = invoke class="VI (strict)" method="Ctrl Val.Set"(reference=w370, error in=w373, "Control Name"="OK", "Value"=TRUE) -> (reference out=w366:refnum<vi>, error out=w368:errorcluster)  [unwired: 1 in, 3 out]
            n135 = call-by-ref "Wait On Asynchronous Call"(reference=w366, error in=w368) -> (reference out=w365:refnum<vi>, error out=w367:errorcluster)  [unwired: 12 in]
            n136 = Close Reference(reference=w365, error in (no error)=w367) -> (error out=w369:errorcluster)
          }
          frame True {
          }
        }
        n137 = call <vilib>:"Clear Errors.vi"("error in (no error)"=w358) -> ("error out"=w355:errorcluster)  [unwired: 5 in, 1 out]
        n138 = call <vilib>:"Add State(s) to Queue__jki_lib_state_machine.vi"("State(s) in (\"\")"=w364) -> ("States Out"=w363:string)  [unwired: 14 in]
      }
      frame "SubPanel: Load" {
        n139 = Unbundle By Name(w382) -> ("VI Ref"=w380:refnum<vi>, "Panel Folder Path"=w384:path, "VI Name"=w383:string, "Time lapse(sec)"=w377:u32)
        n140 = Multiply(x=w377, y=u32 1000) -> (x*y=w375:u32)
        n141 = flat-sequence {
          tunnel: w379 -> [w389]
          tunnel: [w389] -> w378
          tunnel: w375 -> [w388]
          frame #0 {
            n142 = Wait (ms)(milliseconds to wait=w388) -> ()  [unwired: 1 out]
          }
        }
        n143 = case shown="Default" w383 {
          selector: w383 -> [_ w401]
          tunnel: [w391 w397] -> w385
          tunnel: w378 -> [w391 w396]
          tunnel: w384 -> [_ w402]
          tunnel: w382 -> [w390 w400]
          tunnel: [w390 w399] -> w381
          tunnel: w380 -> [_ w392]
          frame "" {
          }
          frame Default {
            n144 = Build Path(base path=w402, name or relative path=w401) -> (appended path=w394:path)
            n145 = File/Directory Info(path=w394, error in=w396) -> (path out=w393:path, error out=w395:errorcluster)  [unwired: 5 out]
            n146 = case shown="No Error" w395 {
              selector: w395 -> [w410 w413]
              tunnel: [w404 _] -> w398
              tunnel: [w406 w412] -> w397
              tunnel: w393 -> [w409 _]
              tunnel: w392 -> [w408 _]
              frame No Error {
                n147 = Open VI Reference(type specifier VI Refnum (for type only)=w408, vi path=w409, options=256, error in (no error)=w410) -> (vi reference=w405:refnum<vi>, error out=w411:errorcluster)  [unwired: 2 in]
                n148 = invoke on="Sub Panel" class="SubPnl" method="Insert VI"(error in=w411, "VI Ref"=w405) -> (error out=w407:errorcluster)  [unwired: 2 in, 3 out]
                n149 = call-by-ref "Start Asynchronous Call"(reference=w405, error in=w407) -> (reference out=w404:refnum<vi>, error out=w406:errorcluster)  [unwired: 12 in]
              }
              frame Error {
                n150 = call <vilib>:"Clear Errors.vi"("error in (no error)"=w413) -> ("error out"=w412:errorcluster)  [unwired: 5 in, 1 out]
              }
            }
            n151 = Bundle By Name(cluster=w400, "VI Ref"=w398) -> (w399:T8)
          }
        }
        n152 = call <vilib>:"Add State(s) to Queue__jki_lib_state_machine.vi"("State(s) in (\"\")"=w387) -> ("States Out"=w386:string)  [unwired: 14 in]
      }
      frame "SubPanel 2: Unload" {
        n153 = invoke on="Sub Panel 2" class="SubPnl" method="Remove VI"(error in=w419) -> (error out=w417:errorcluster)  [unwired: 2 in, 2 out]
        n154 = Unbundle By Name(w418) -> ("Panel 2 VI ref"=w415:refnum<vi>)
        n155 = Not A Number/Path/Refnum?(number/path/refnum=w415) -> (NaN/Path/Refnum?=w414:bool)
        n156 = case shown="True" w414 {
          tunnel: w415 -> [w423 _]
          tunnel: w417 -> [w422 w424]
          tunnel: [w421 w424] -> w416
          frame False {
            n157 = Close Reference(reference=w423, error in (no error)=w422) -> (error out=w421:errorcluster)
          }
          frame True {
          }
        }
      }
      frame "SubPanel 2: Load" {
        n158 = Unbundle By Name(w426) -> ("Panel 2 Folder Path"=w432:path, "VI Name"=w433:string)
        n159 = Build Path(base path=w432, name or relative path=w433) -> (appended path=w431:path)
        n160 = Open VI Reference(vi path=w431, error in (no error)=w429) -> (vi reference=w427:refnum<vi>, error out=w430:errorcluster)  [unwired: 4 in]
        n161 = invoke on="Sub Panel 2" class="SubPnl" method="Insert VI"(error in=w430, "VI Ref"=w427) -> (error out=w428:errorcluster)  [unwired: 2 in, 3 out]
        n162 = Bundle By Name(cluster=w426, "Panel 2 VI ref"=w427) -> (w425:T8)
      }
      frame "---------------Run------------" {
      }
      frame "Run VI" {
        n163 = in-place {
          in-place-border: w441 -> [w447]
          in-place-border: [w446] -> w439
          n164 = in-place-cluster #1(w440) -> ("Panel 2 VI ref"=w445:refnum<vi>)  [unwired: 1 out]
          n165 = invoke class="VI" method="Run VI"(reference=w445, error in=w447, "Wait until done"=FALSE ("Wait Until Done"), "Auto Dispose Ref"=FALSE ("Auto Dispose Reference")) -> (reference out=w444:refnum<vi>, error out=w446:errorcluster)  [unwired: 1 in, 3 out]
          n166 = in-place-cluster #1("VI Running?"=TRUE, "Panel 2 VI ref"=w444) -> (w438:T8)
        }
      }
      frame "---------- New Category ----------" {
        # "Template Separator\n(You can make a copy of, or modify, this frame)"
        n167 = call <vilib>:"Add State(s) to Queue__jki_lib_state_machine.vi"("State(s) in (\"\")"=w453) -> ("States Out"=w452:string)  [unwired: 14 in]
      }
      frame "New Category: 2" {
        # "Your code here.\n(You can make a copy of, or modify, this frame)"
        n168 = call <vilib>:"Add State(s) to Queue__jki_lib_state_machine.vi"("State(s) in (\"\")"=w457) -> ("States Out"=w456:string)  [unwired: 14 in]
      }
    }
  }
